vi "Multi VI Demo.vi"(0 "N":i32=5) -> (1 "Sum":i32, 2 "Count":i32, 3 "Mean":dbl)   [LabVIEW 2026]
doc: "Round20 P6 flagship: a top-level VI orchestrating two subVIs through Call nodes - Accumulate N.vi (While Loop + 2 shift registers, Sum/Count) and Mean Of Pair.vi (Divide). Data crosses connector panes twice: N in, Sum/Count/Mean out. Expected outputs, hand-computed: N=5 gives Sum=15, Count=5, Mean=3.0; N=3 gives Sum=6, Count=3, Mean=2.0. The int-to-DBL promotion happens inside Mean Of Pair and crosses the caller's pane as DBL. Call output net ids are their own numbers (not the Call node's uid), per the round-6 recipe."
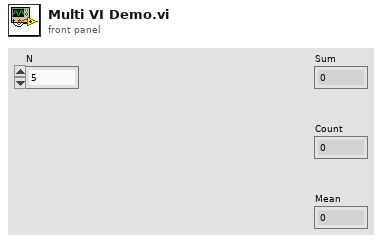
[diagram p1: front panel]
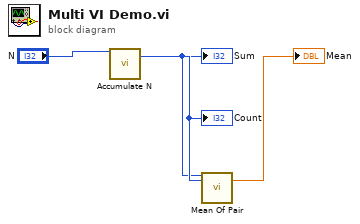
[diagram p0: block diagram]
diagram:
  n1 = call "Accumulate N.vi"("N"="N") -> ("Sum"=w2:i32, "Count"=w3:i32)  [unwired: 13 in]
  "Sum" <- w2
  "Count" <- w3
  n2 = call "Mean Of Pair.vi"("x"=w2, "y"=w3) -> ("Mean"=→"Mean":dbl)  [unwired: 13 in]
